vi "UMLEditor drawGrabbers.vi"(1 "graphics":refnum<class "Graphics.lvclass">, 2 "points":T1[](array[typedef]) {"y" format="%.2f"; "x" format="%.2f"}, 5 "error in (no error)":errorcluster) -> (15 "picture":picture, 19 "error out":errorcluster)   [LabVIEW 2020]
doc: "Draws grabbers"
uses:
  <resource>/Framework/Providers/Open_GDS/UML/General/Point/Point Point2D.ctl
  <resource>/Framework/Providers/Open_GDS/UML/Graphics_class/Graphics.lvclass
  <resource>/Framework/Providers/Open_GDS/UML/General/Rectangle/Rectangle Rectangle2D.ctl
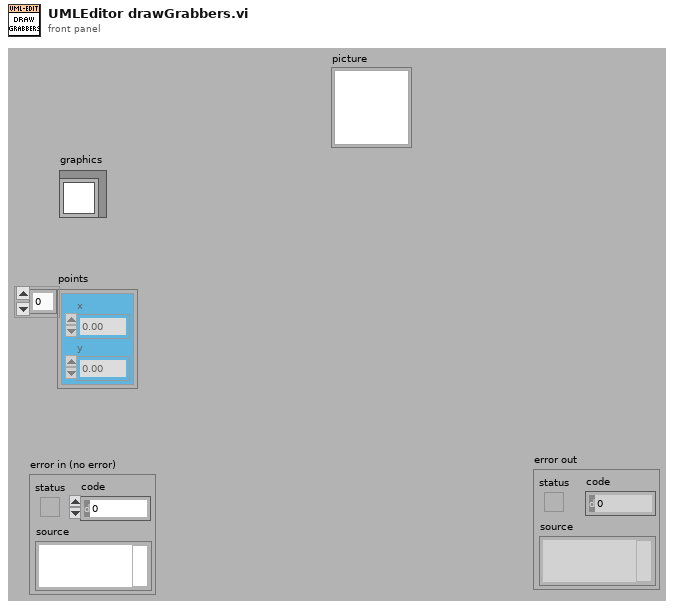
[diagram p1: front panel]
types:
  T1 = typedef "Point Point2D.ctl" = cluster{"x":dbl, "y":dbl}
  T2 = typedef "Rectangle Rectangle2D.ctl" = cluster{"x":dbl, "y":dbl, "width":dbl, "height":dbl}
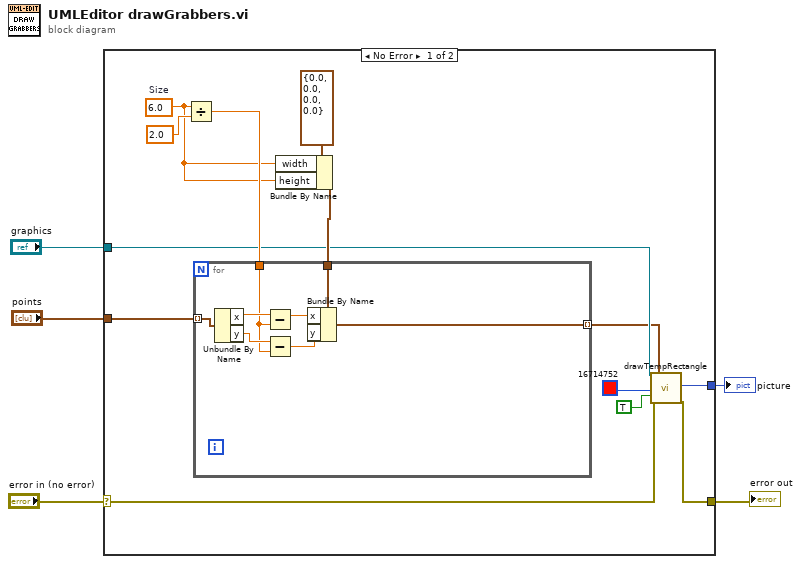
[diagram p0: block diagram]
diagram:
  n1 = case shown="No Error" "error in (no error)" {
    selector: "error in (no error)" -> [w8 w27]
    tunnel: [w7 w27] -> w4
    tunnel: "graphics" -> [w10 _]
    tunnel: "points" -> [w18 _]
    tunnel: [w6 _] -> w1
    frame No Error {
      w14 = 6.0  # Size
      n2 = Divide(x=w14, y=2.0) -> (x/y=w16:dbl)
      n3 = Bundle By Name(cluster=T2 {"x"=0.0, "y"=0.0, "width"=0.0, "height"=0.0} ("rectangle"), "width"=w14, "height"=w14) -> (w13:T2)
      n4 = for {
        tunnel: w18 -> [w26] mode=indexing
        tunnel: w16 -> [w23]
        tunnel: w13 -> [w22]
        tunnel: [w19] -> w9 mode=indexing
        n5 = Unbundle By Name(w26) -> ("x"=w25:dbl, "y"=w24:dbl)
        n6 = Subtract(x=w25, y=w23) -> (x-y=w21:dbl)
        n7 = Subtract(x=w24, y=w23) -> (x-y=w20:dbl)
        n8 = Bundle By Name(cluster=w22, "x"=w21, "y"=w20) -> (w19:T2)
      }
      n9 = call <resource>:"drawTempRectangle.vi"("reference"=w10, "color(if not used=default color)"=u32 16714752, "fill?(F)"=TRUE, "error in (no error)"=w8, "Rectangles"=w9) -> ("picture"=w6:picture, "error out"=w7:errorcluster)  [unwired: 3 in, 10 out]
    }
    frame Error {
    }
  }
  "error out" <- w4
  "picture" <- w1
